vi "TI_Proyecto3_ultimo1_conMyDAQ.vi"() -> ()   [LabVIEW 2025]
uses:
  <vilib>/measure/NI_MABase.lvlib
panel:
  in  "String":string
  in  "Path":path
  out "Delay":dbl
  out "Waveform Chart":dynamicdata(graph)
  out "Senoidal Salida":dbl[](array[numeric])
  out "Salida DAC":dbl
  out "Valor entrada DAC":u32
  out "Entrada DAC":bool[](array[boolean])
  out "Salida SPI":i16[](array[numeric])
  out "Entrada SPI":i16[](array[numeric])
  out "reversed array":bool[](array[boolean])
  out "Valor binario":dbl
  out "Valor de la muestra":dbl
  out "Waveform Chart 2":dynamicdata(graph)
  out "Waveform Graph 2":dynamicdata(graph)
  in  "signal type":T1(ring)
  in  "sampling info":cluster{"Fs":dbl, "#s":dbl}={"Fs"=1000.0, "#s"=1000.0} {"Fs" format="%.2p"}
  out "Waveform Graph":waveform(dbl)(graph)
  out "Muestra actual":dbl
  out "Señal senoidal":dbl[](array[numeric])
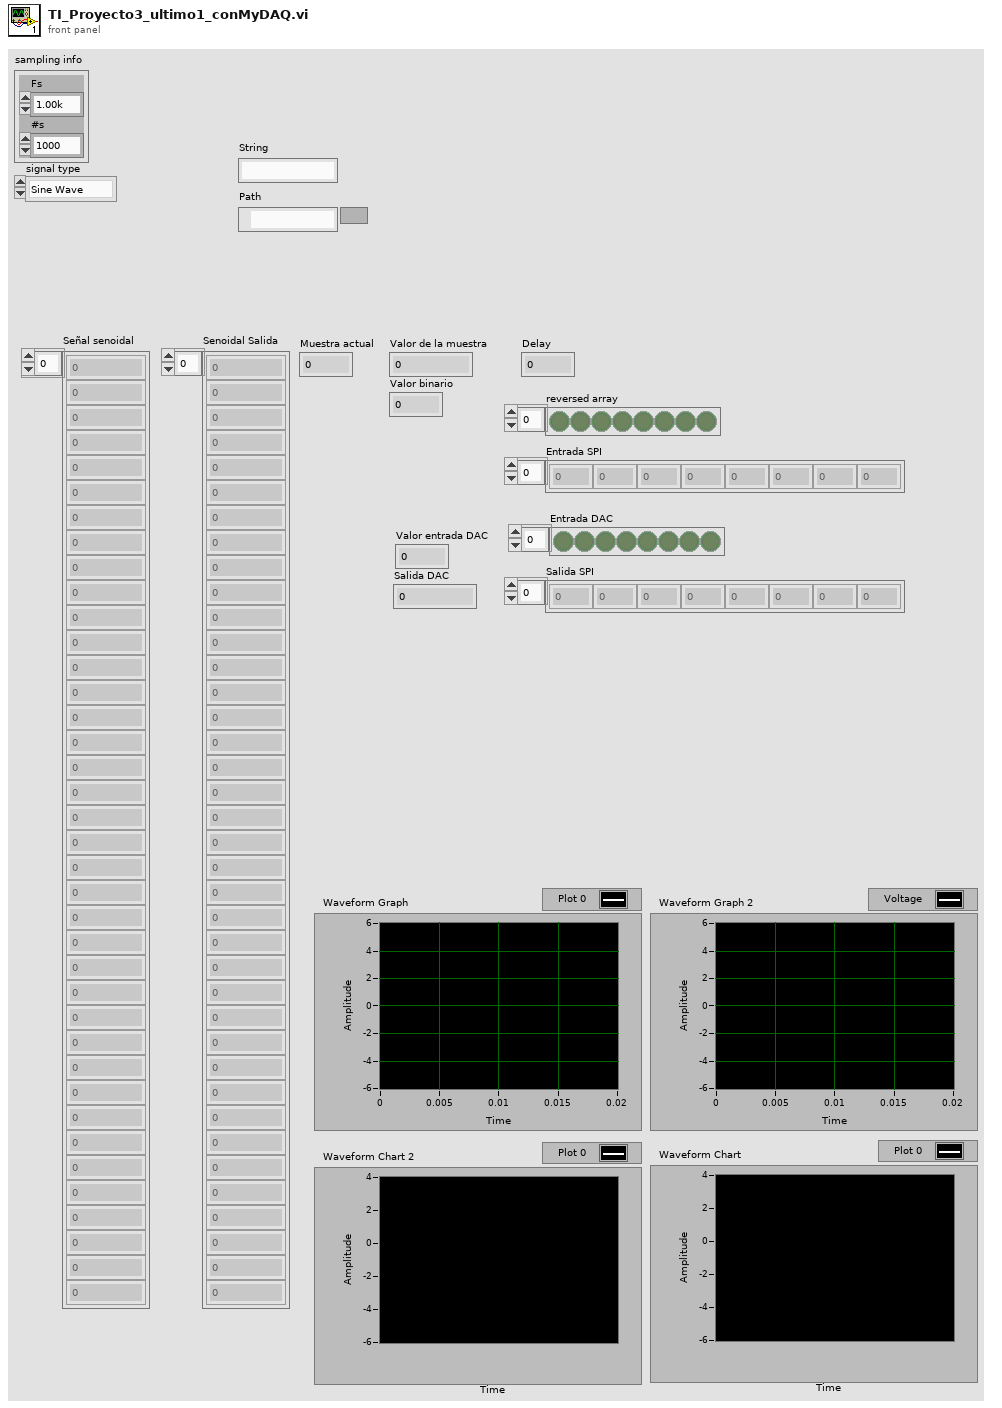
[diagram p1: front panel]
types:
  T1 = enum16{"Sine Wave", "Triangle Wave", "Square Wave", "Sawtooth Wave"}
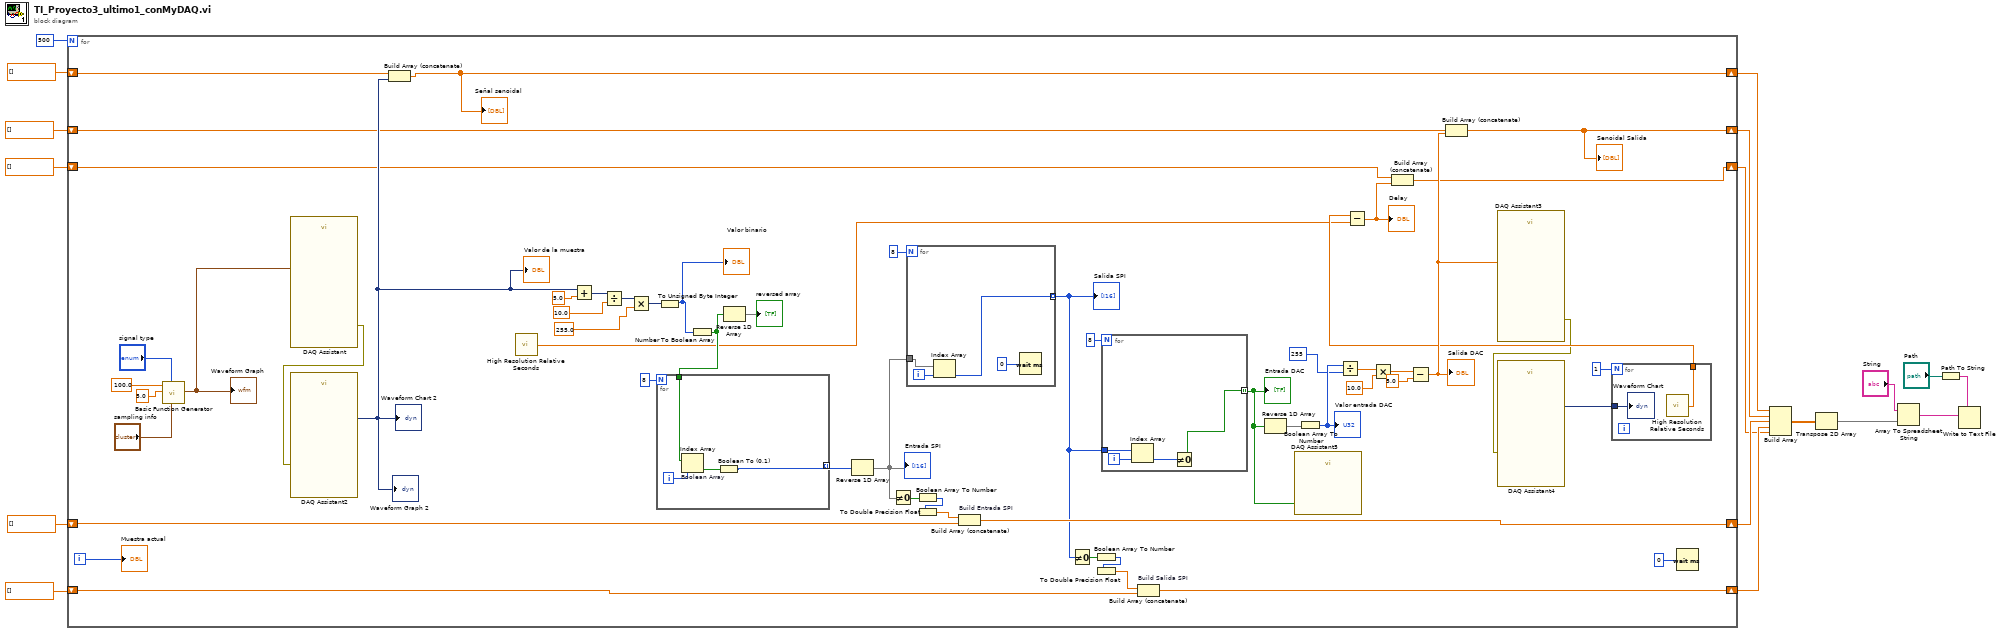
[diagram p0: block diagram]
diagram:
  n1 = for {
    N: 500 -> [_]
    shift-right: [w67] -> w7
    shift-left: dbl[] [] -> [w66]
    shift-right: [w33] -> w8
    shift-left: dbl[] [] -> [w34]
    shift-right: [w31] -> w5
    shift-left: dbl[] [] -> [w32]
    shift-right: [w21] -> w3
    shift-left: dbl[] [] -> [w22]
    shift-right: [w18] -> w1
    shift-left: dbl[] [] -> [w19]
    i -> [w64]
    n2 = call <vilib>:"Basic Function Generator.vi"("sampling info"="sampling info", "signal type"="signal type", "amplitude"=5.0, "frequency"=100.0) -> ("signal out"=w69:waveform(dbl))  [unwired: 5 in, 2 out]
    "Waveform Graph" <- w69
    n3 = call "DAQ Assistant"("data"=w69) -> ("error out"=w35:errorcluster)  [unwired: 17 in, 1 out]
    n4 = call "DAQ Assistant2"("error in"=w35) -> ("data"=w37:dynamicdata)  [unwired: 16 in, 2 out]
    "Waveform Graph 2" <- w37
    "Waveform Chart 2" <- w37
    "Valor de la muestra" <- w37
    n5 = Build Array (concatenate) "Build Array"(w66, w37) -> (w67:dbl[])
    "Señal senoidal" <- w67
    n6 = call <vilib>:"High Resolution Relative Seconds.vi"() -> ("relative seconds"=w38:dbl)
    n7 = Add(x=w37, y=5.0) -> (x+y=w62:dynamicdata)
    n8 = Divide(x=w62, y=10.0) -> (x/y=w60:dynamicdata)
    n9 = Multiply(x=w60, y=255.0) -> (x*y=w58:dynamicdata)
    n10 = To Unsigned Byte Integer(number=w58) -> (unsigned 8bit integer=w57:u8)
    "Valor binario" <- w57
    n11 = Number To Boolean Array(number=w57) -> (Boolean array=w54:bool[])
    n12 = for {
      N: 8 -> [_]
      tunnel: w54 -> [w83]
      tunnel: [w84] -> w53 mode=indexing
      i -> [w85]
      n13 = Index Array "Boolean Array"(array=w83, index=w85) -> (element=w86:bool)
      n14 = Boolean To (0,1)(Boolean=w86) -> (0, 1=w84:i16)
    }
    n15 = Reverse 1D Array(array=w54) -> (reversed array=→"reversed array":bool[])
    n16 = Reverse 1D Array(array=w53) -> (reversed array=w29:i16[])
    "Entrada SPI" <- w29
    n17 = Not Equal To 0?(x=w29) -> (x != 0?=w27:bool[])
    n18 = for {
      N: 8 -> [_]
      tunnel: w29 -> [w81]
      tunnel: [w79] -> w24 mode=indexing
      i -> [w82]
      n19 = Index Array(array=w81, index=w82) -> (element=w79:i16)
      n20 = Wait (ms)(milliseconds to wait=u32 0) -> ()  [unwired: 1 out]
    }
    "Salida SPI" <- w24
    n21 = Boolean Array To Number(Boolean array=w27) -> (number=w28:u32)
    n22 = To Double Precision Float(number=w28) -> (double precision float=w30:dbl)
    n23 = Build Array (concatenate) "Build Entrada SPI"(w30, w32) -> (w31:dbl[])
    n24 = Not Equal To 0?(x=w24) -> (x != 0?=w25:bool[])
    n25 = Boolean Array To Number(Boolean array=w25) -> (number=w23:u32)
    n26 = To Double Precision Float(number=w23) -> (double precision float=w26:dbl)
    n27 = for {
      N: 8 -> [_]
      tunnel: w24 -> [w77]
      tunnel: [w75] -> w42 mode=indexing
      i -> [w78]
      n28 = Index Array(array=w77, index=w78) -> (element=w76:i16)
      n29 = Not Equal To 0?(x=w76) -> (x != 0?=w75:bool)
    }
    "Entrada DAC" <- w42
    n30 = Build Array (concatenate) "Build Salida SPI"(w26, w22) -> (w21:dbl[])
    n31 = Reverse 1D Array(array=w42) -> (reversed array=w50:bool[])
    n32 = call "DAQ Assistant5"("data"=w42) -> ()  [unwired: 17 in, 2 out]
    n33 = Boolean Array To Number(Boolean array=w50) -> (number=w45:u32)
    "Valor entrada DAC" <- w45
    n34 = Divide(x=w45, y=u32 255) -> (x/y=w49:dbl)
    n35 = Multiply(x=w49, y=10.0) -> (x*y=w47:dbl)
    n36 = Subtract(x=w47, y=5.0) -> (x-y=w43:dbl)
    "Salida DAC" <- w43
    n37 = Build Array (concatenate) "Build Array"(w34, w43) -> (w33:dbl[])
    "Senoidal Salida" <- w33
    n38 = call "DAQ Assistant3"("data"=w43) -> ("error out"=w36:errorcluster)  [unwired: 17 in, 1 out]
    n39 = call "DAQ Assistant4"("error in"=w36) -> ("data"=w40:dynamicdata)  [unwired: 16 in, 2 out]
    n40 = for {
      N: u32 1 ("milliseconds to wait") -> [_]
      tunnel: w40 -> [w74]
      tunnel: [w73] -> w39
      n41 = call <vilib>:"High Resolution Relative Seconds.vi"() -> ("relative seconds"=w73:dbl)
      "Waveform Chart" <- w74
    }
    n42 = Subtract(x=w39, y=w38) -> (x-y=w20:dbl)
    "Delay" <- w20
    n43 = Build Array (concatenate)(w19, w20) -> (w18:dbl[])
    n44 = Wait (ms)(milliseconds to wait=u32 0) -> ()  [unwired: 1 out]
    "Muestra actual" <- w64
  }
  n45 = Build Array "Build Array"(w7, w8, w5, w3, w1) -> (w10:dbl[][])
  n46 = Transpose 2D Array(2D array=w10) -> (transposed array=w9:dbl[][])
  n47 = Array To Spreadsheet String(array=w9, 3:"String") -> (spreadsheet string=w11:string)  [unwired: 1 in]
  n48 = Path To String(path="Path") -> (string=w13:string)
  n49 = Write to Text File(prompt (Choose or enter file path)=w13, text=w11) -> ()  [unwired: 2 in, 3 out]
